vi "Get User FullName.vi"(4 "error in (no error)":errorcluster, 6 "LoginName":string, 7 "EasyUserManager in":refnum<class "EasyUserManager.lvclass">) -> (0 "error out":errorcluster, 1 "FullName":string, 3 "EasyUserManager out":refnum<class "EasyUserManager.lvclass">)   [LabVIEW 2024, in "EasyUserManager.lvclass"]
doc: "Get the <B>FullName</B> of the user specified by <B>LoginName</B>."
uses:
  EasyUserManager.lvclass
  EasyUserManager.lvclass/EasyUserManager.ctl
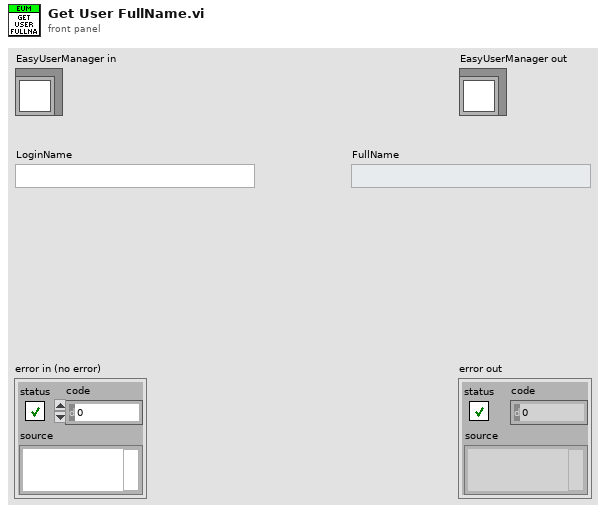
[diagram p1: front panel]
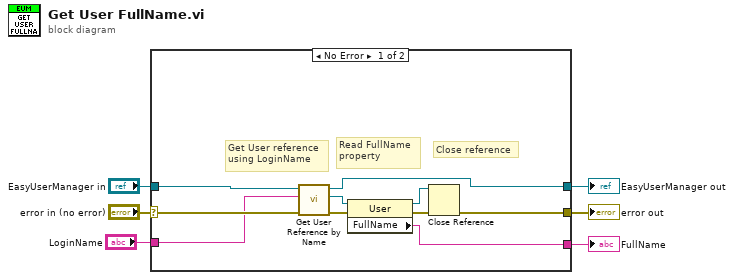
[diagram p0: block diagram]
diagram:
  n1 = case shown="No Error" "error in (no error)" {
    selector: "error in (no error)" -> [w9 w18]
    tunnel: [w10 w18] -> w5
    tunnel: [w11 w17] -> w3
    tunnel: "EasyUserManager in" -> [w16 w17]
    tunnel: "LoginName" -> [w8 _]
    tunnel: [w7 _] -> w1
    frame No Error {
      # "Close reference"
      # "Read FullName\nproperty"
      # "Get User reference \nusing LoginName"
      n2 = call "Get User Reference by Name.vi"("error in (no error)"=w9, "LoginName"=w8, "EasyUserManager in"=w16) -> ("error out"=w14:errorcluster, "User Reference"=w15:refnum<k7>, "EasyUserManager out"=w11:refnum<class "EasyUserManager.lvclass">)  [unwired: 2 in]
      n3 = property on="Property Node" class="User"(reference=w15, error in=w14) -> (reference out=w13:refnum<k7>, error out=w12:errorcluster, "FullName"=w7:string)
      n4 = Close Reference(reference=w13, error in (no error)=w12) -> (error out=w10:errorcluster)
    }
    frame Error {
      # "Pass error and do nothing."
    }
  }
  "error out" <- w5
  "EasyUserManager out" <- w3
  "FullName" <- w1
